vi "motor_control.vi"() -> ()   [LabVIEW 2026]
panel:
  out "Invert X":bool
  in  "Motor Clock Num per Pulse":u32=100
  in  "Port0 Bits":tag="Dev1/port0/line0:7"
  in  "Laser Sync Source":tag="/Dev1/PFI8"
  in  "Laser DO Rate":u32=40000
  in  "Motor Pulse Rate":i32=200
  in  "kx":dbl=1.0
  in  "Move X":bool
  in  "delta_x":dbl=1.0
  in  "xdir":bool=TRUE
  # "mm"
  # "mm/s"
  # "(steps/mm)"
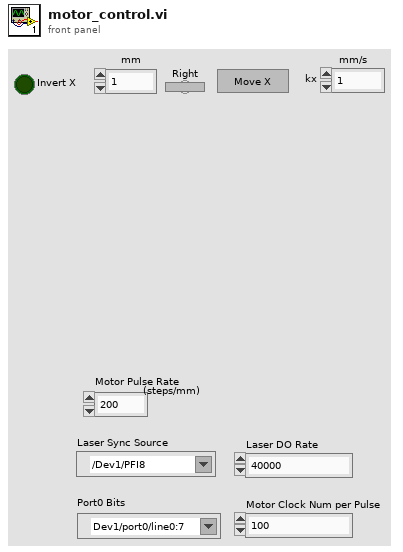
[diagram p1: front panel]
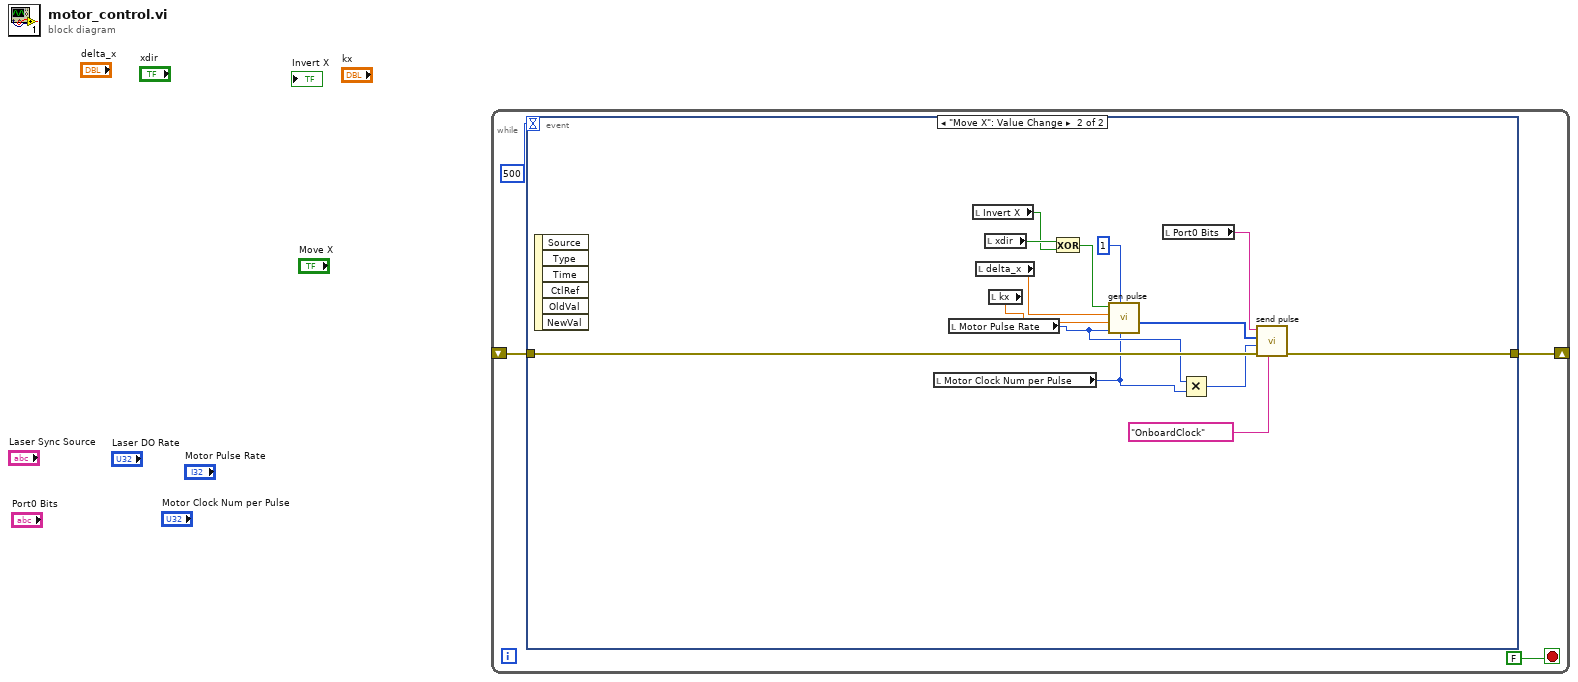
[diagram p0: block diagram]
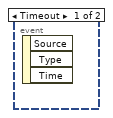
[diagram p2: hidden frame]
diagram:
  n1 = while {
    shift-right: [w3] -> _
    shift-left: _ -> [w2]
    stop <- FALSE stop-if-true
    n2 = event shown="[1] \"Move X\": Value Change" {
      selector: _ -> [_ _]
      dyn-events: _ -> [_ _]
      timeout: 500 -> [_ _]
      tunnel: [_ w18] -> w3
      tunnel: w2 -> [_ w17]
      event Timeout {
        n3 = event-data() -> ()  [unwired: 1 in, 3 out]
      }
      event "Move X": Value Change {
        n4 = event-data() -> ()  [unwired: 1 in, 6 out]
        n5 = local read "Motor Clock Num per Pulse"() -> (w10:u32)
        n6 = local read "Motor Pulse Rate"() -> (w11:i32)
        n7 = local read "Invert X"() -> (w5:bool)
        n8 = local read "delta_x"() -> (w15:dbl)
        n9 = local read "xdir"() -> (w7:bool)
        n10 = local read "kx"() -> (w14:dbl)
        n11 = Exclusive Or(1:w5, 2:w7) -> (0:w6:bool)
        n12 = call "gen pulse.vi"("clk per pulse"=w10, "bit"=u8 1, "Motor Pulse Rate / mm"=w11, "kx"=w14, "xn"=w15, "dir"=w6) -> ("pulsetrain"=w13:u8[])  [unwired: 3 in, 2 out]
        n13 = local read "Port0 Bits"() -> (w12:tag)
        n14 = Multiply(x=w11, y=w10) -> (x*y=w9:u32)
        n15 = call "send pulse.vi"("source"=tag "OnboardClock", "error in"=w17, "Motors DO rate"=w9, "P0 DO data"=w13, "Port0 Bits"=w12) -> ("error out"=w18:errorcluster)  [unwired: 6 in]
      }
    }
  }
